vi "OpenCycle.vi"(0 "PLC":refnum<vi>) -> ()   [LabVIEW 2023]
uses:
  S7Plc.ctl
  D:/Projects/S7View/S7Lib/bin/Debug/S7.Net.dll
  S7Lib/bin/Debug/S7.Net.dll
  D:/Projects/S7View/S7Lib/bin/Debug/S7Lib.dll
  S7Lib/bin/Debug/S7Lib.dll
panel:
  out "错误输出":errorcluster
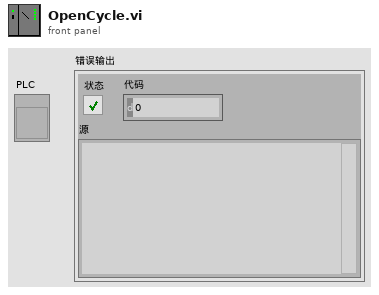
[diagram p1: front panel]
types:
  T1 = typedef "S7Plc.ctl" = cluster{"ip":string, "type":i16, "rack":i16, "slot":i16, "status":bool, "link":bool, "c_msg":string, "r_msg":string, "w_msg":string, "plc":refnum<k24>, "ok":bool}
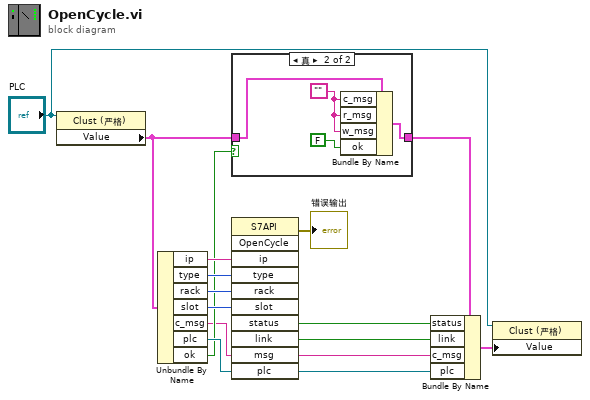
[diagram p0: block diagram]
diagram:
  n1 = property on="属性节点" class="Clust (严格)"(reference="PLC") -> ("Value"=w3:T1)  [unwired: 1 in, 2 out]
  n2 = Unbundle By Name(w3) -> ("ip"=w16:string, "type"=w15:i16, "rack"=w14:i16, "slot"=w13:i16, "c_msg"=w1:string, "plc"=w9:refnum<k24>, "ok"=w4:bool)
  n3 = case shown="真" w4 {
    tunnel: w3 -> [w17 w21]
    tunnel: [w17 w20] -> w2
    frame False {
    }
    frame True {
      w19 = ""
      n4 = Bundle By Name(cluster=w21, "c_msg"=w19, "r_msg"=w19, "w_msg"=w19, "ok"=FALSE) -> (w20:T1)
    }
  }
  n5 = invoke on="调用节点" class="S7API" method="OpenCycle"("ip"=w16, "type"=w15, "rack"=w14, "slot"=w13, "msg"=w1, "plc"=w9) -> (error out=→"错误输出":errorcluster, "status"=w8:bool, "link"=w7:bool, "msg"=w6:string, "plc"=w5:refnum<k24>)  [unwired: 5 in, 6 out]
  n6 = Bundle By Name(cluster=w2, "status"=w8, "link"=w7, "c_msg"=w6, "plc"=w5) -> (w12:T1)
  n7 = property on="属性节点" class="Clust (严格)"(reference="PLC", "Value"=w12) -> ()  [unwired: 1 in, 2 out]
